vi "Enumerate User Inputs.vi"(8 "error in":errorcluster, 11 "User Input Collection":T1) -> (0 "error out":errorcluster, 3 "Entries":cluster{"Key":string, "Value":string}[](array[cluster]))   [LabVIEW 2026, in "ToastNotification.lvlib" / "ToastService.lvclass"]
doc: "Enumerate a borrowed UserInput collection and copy all entries into LabVIEW key/value pairs. Null collection returns an empty array. Acquire an enumerator, call MoveNext before reading Current, release boxed iteration results, dispose when supported, and close the enumerator on success and failure. Do not close the collection here. Stop at the first error and retain entries already copied."
uses:
  ToastService.lvclass
  Reflection DotNet/Callback Object Reference.ctl
  Reflection DotNet/Reflection DotNet.lvlib
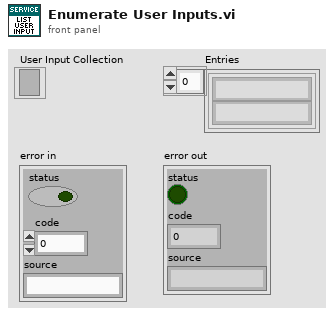
[diagram p1: front panel]
types:
  T1 = typedef "ToastNotification.lvlib/Reflection DotNet.lvlib/Callback Object Reference.ctl" = refnum<k24>
  T2 = typedef "ToastNotification.lvlib/Argument.ctl" = cluster{"Key":string, "Value":string}
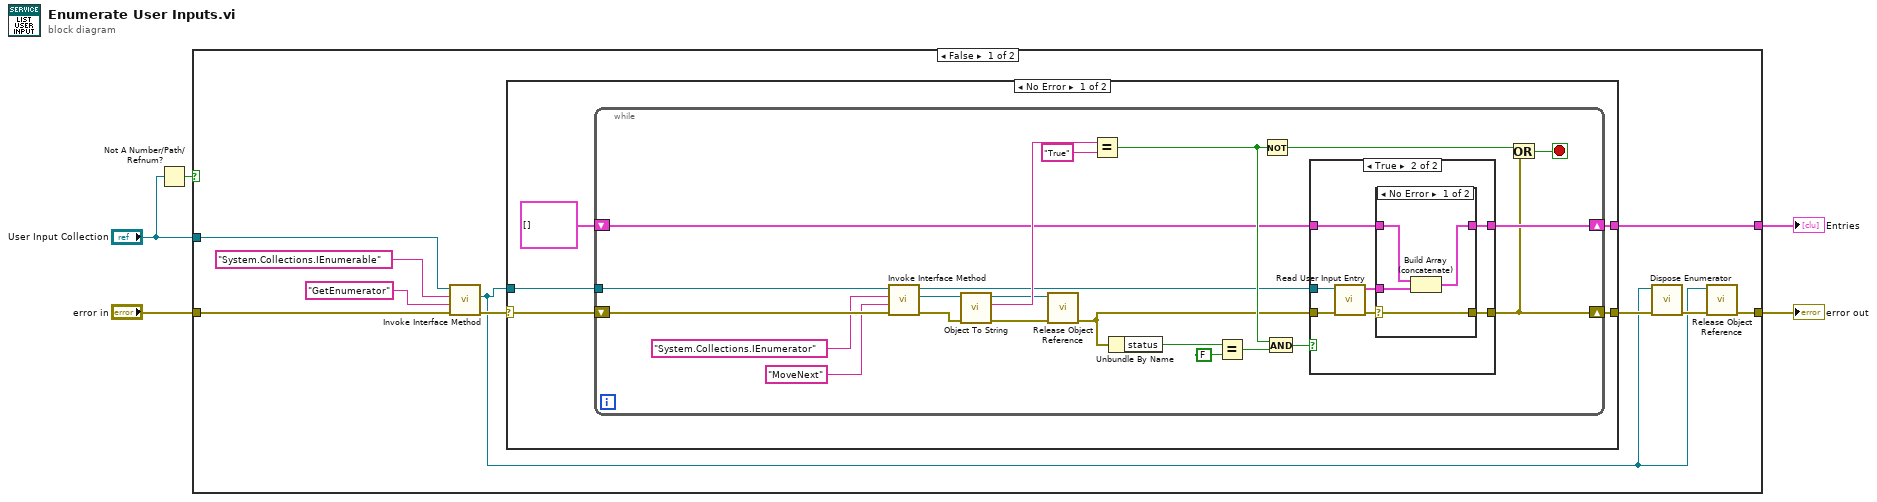
[diagram p0: block diagram]
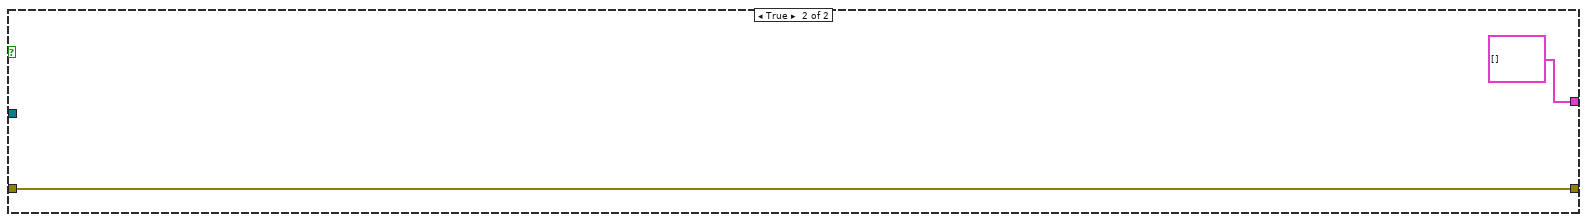
[diagram p5: hidden frame]
diagram:
  n1 = Not A Number/Path/Refnum?(number/path/refnum="User Input Collection") -> (NaN/Path/Refnum?=w3:bool)
  n2 = case shown="False" w3 {
    tunnel: "User Input Collection" -> [w11 _]
    tunnel: "error in" -> [w8 w60]
    tunnel: [w12 cluster{"Key":string, "Value":string}[] []] -> w4
    tunnel: [w15 w60] -> w5
    frame False {
      n3 = call "Invoke Interface Method.vi"("error in"=w8, "method name"="GetEnumerator", "interface name"="System.Collections.IEnumerable", "object in"=w11) -> ("error out"=w7:errorcluster, "value"=w6:T1)  [unwired: 5 in, 1 out]
      n4 = case shown="No Error" w7 {
        selector: w7 -> [w16 w58]
        tunnel: [w20 cluster{"Key":string, "Value":string}[] []] -> w12
        tunnel: w6 -> [w17 _]
        tunnel: [w18 w58] -> w13
        frame No Error {
          n5 = while {
            shift-right: [w31] -> w20
            shift-left: cluster{"Key":string, "Value":string}[] [] -> [w30]
            shift-right: [w26] -> w18
            shift-left: w16 -> [w29]
            tunnel: w17 -> [w23]
            stop <- w42 stop-if-true
            n6 = call "Invoke Interface Method.vi"("error in"=w29, "method name"="MoveNext", "interface name"="System.Collections.IEnumerator", "object in"=w23) -> ("error out"=w27:errorcluster, "value"=w22:T1, "object out"=w24:T1)  [unwired: 5 in]
            n7 = call "Object To String.vi"("error in (no error)"=w27, "Object in"=w22) -> ("error out"=w33:errorcluster, "Text"=w32:string, "Object out"=w21:refnum<k24>)  [unwired: 7 in]
            n8 = call "Release Object Reference.vi"("error in"=w33, "object"=w21) -> ("error out"=w34:errorcluster)  [unwired: 9 in]
            n9 = Equal?(x=w32, y="True") -> (x = y?=w36:bool)
            n10 = Unbundle By Name(w34) -> ("status"=w37:bool)
            n11 = Equal?(x=w37, y=FALSE) -> (x = y?=w39:bool)
            n12 = Not(x=w36) -> (.not. x?=w41:bool)
            n13 = And(x=w36, y=w39) -> (x .and. y?=w40:bool)
            n14 = case shown="True" w40 {
              tunnel: w30 -> [w44 w47]
              tunnel: w24 -> [_ w45]
              tunnel: w34 -> [w43 w46]
              tunnel: [w43 w51] -> w26
              tunnel: [w44 w50] -> w31
              frame False {
              }
              frame True {
                n15 = call "Read User Input Entry.vi"("error in"=w46, "User Input Enumerator"=w45) -> ("error out"=w49:errorcluster, "Entry"=w48:T2)  [unwired: 8 in]
                n16 = case shown="No Error" w49 {
                  selector: w49 -> [w52 w56]
                  tunnel: w47 -> [w53 w57]
                  tunnel: w48 -> [w54 _]
                  tunnel: [w52 w56] -> w51
                  tunnel: [w55 w57] -> w50
                  frame No Error {
                    n17 = Build Array (concatenate)(w53, w54) -> (w55:T2[])
                  }
                  frame Error {
                  }
                }
              }
            }
            n18 = Or(x=w41, y=w26) -> (x .or. y?=w42:bool)
          }
        }
        frame Error {
        }
      }
      n19 = call "Dispose Enumerator.vi"("error in"=w13, "Enumerator"=w6) -> ("error out"=w14:errorcluster)  [unwired: 9 in]
      n20 = call "Release Object Reference.vi"("error in"=w14, "object"=w6) -> ("error out"=w15:errorcluster)  [unwired: 9 in]
    }
    frame True {
    }
  }
  "Entries" <- w4
  "error out" <- w5
